vi "DisplayImage.vi"(0 "image color":T2, 1 "Image Pixel Data":u32[](array[numeric]), 3 "data type":T4(ring), 5 "Image grayscale":T2, 9 "width":u16, 11 "error in (no error)":errorcluster, 12 "height":u16, 13 "interpretation":T3(ring), 14 "bayer parameters":T1) -> (4 "display image":T2, 15 "error out":errorcluster)   [LabVIEW 2025, in "Automotive Vision UI.lvlib"]
doc: "Transform the received picture pixels to an actual image based on the image type."
uses:
  <vilib>/vision/Image Controls.llb/IMAQ Image.ctl
  Automotive Vision UI.lvlib
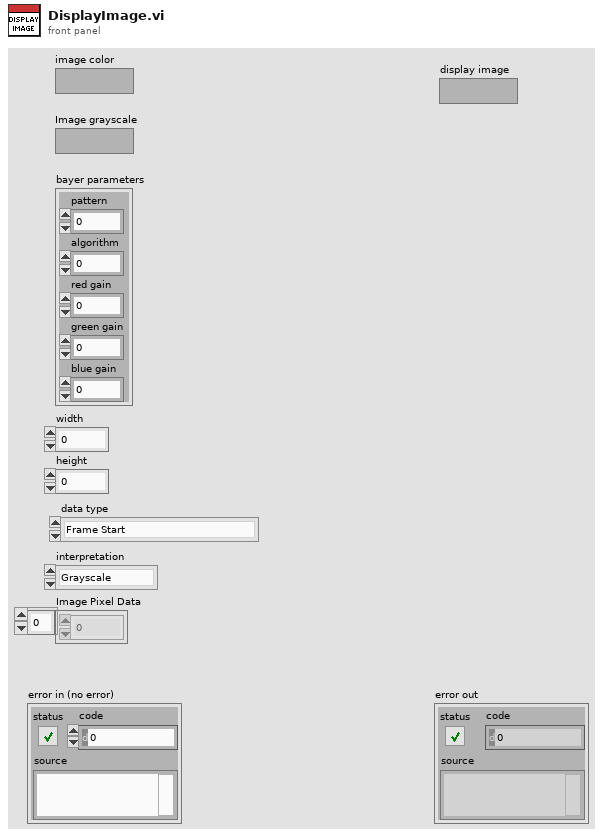
[diagram p1: front panel]
types:
  T1 = cluster{"pattern":i32, "algorithm":i32, "red gain":dbl, "green gain":dbl, "blue gain":dbl}
  T2 = typedef "IMAQ Image.ctl" = refnum<image>
  T3 = enum16{"Grayscale", "Bayer", "RGB", "YUV422", "YUV420", "Legacy YUV420"}
  T4 = enum8{"Frame Start", "Frame End", "Line Start", "Line End", "End of Transmission", "Reserved 0", "Reserved 1", "Reserved 2", "Generic Short Packet 1", "Generic Short Packet 2", "Generic Short Packet 3", "Generic Short Packet 4", "Generic Short Packet 5", "Generic Short Packet 6", "Generic Short Packet 7", "Generic Short Packet 8", "Null", "Blanking Data", "Embedded 8-bit non Image Data", "Generic Long Packet 1", "Generic Long Packet 2", "Generic Long Packet 3", "Generic Long Packet 4", "Reserved 3", "YUV420 8-bit", "YUV420 10-bit", "Legacy YUV420 8-bit", "Reserved 4", "YUV420 8-bit Chroma Shifted", "YUV420 10-bit Chroma Shifted", "YUV422 8-bit", "YUV422 10-bit", "RGB444", "RGB555", "RGB565", "RGB666", "RGB888", "Reserved 5", "Reserved 6", "RAW 24", "RAW 6", "RAW 7", "RAW 8", "RAW 10", "RAW 12", "RAW 14", "RAW 16", "RAW 20", "User Defined 8-bit Data 1", "User Defined 8-bit Data 2", "User Defined 8-bit Data 3", "User Defined 8-bit Data 4", "User Defined 8-bit Data 5", "User Defined 8-bit Data 6", "User Defined 8-bit Data 7", "User Defined 8-bit Data 8", "USL Command", "Reserved 7", "Reserved 8", "Reserved 9", "Reserved 10", "Reserved 11", "Reserved 12", "LRTE EPD Spacer"}
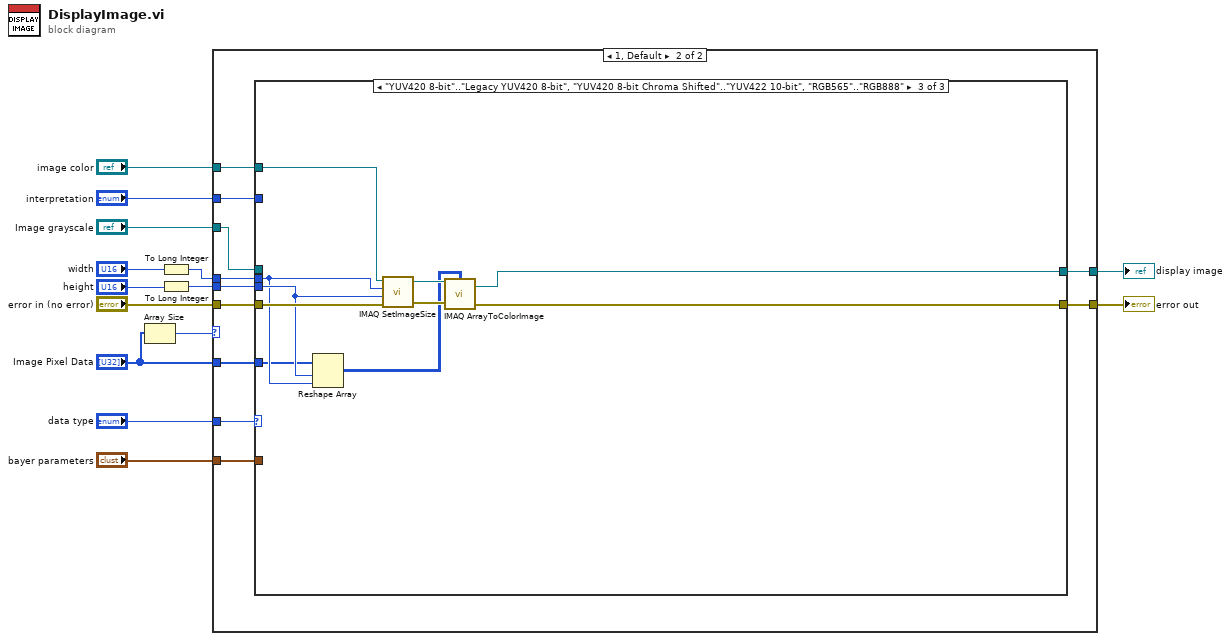
[diagram p0: block diagram]
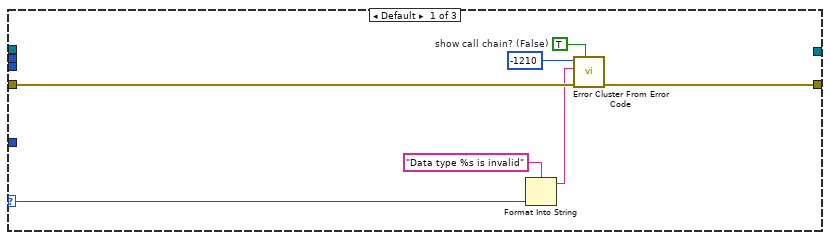
[diagram p3: hidden frame]
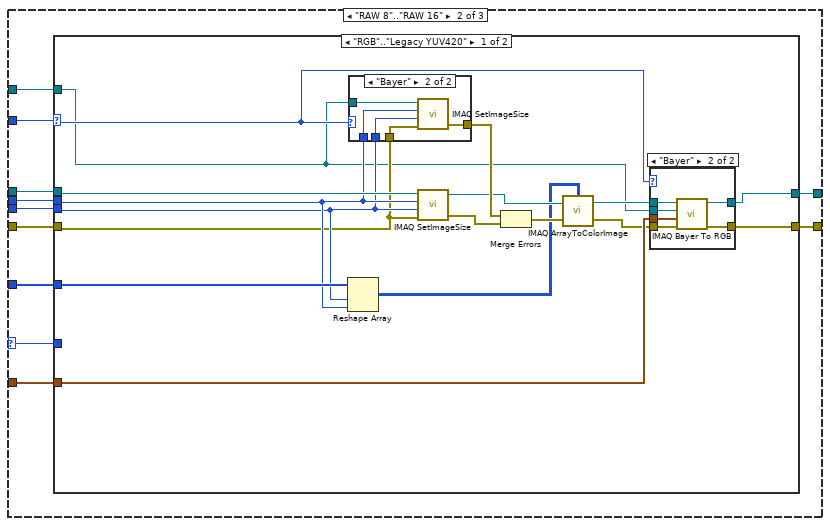
[diagram p4: hidden frame]
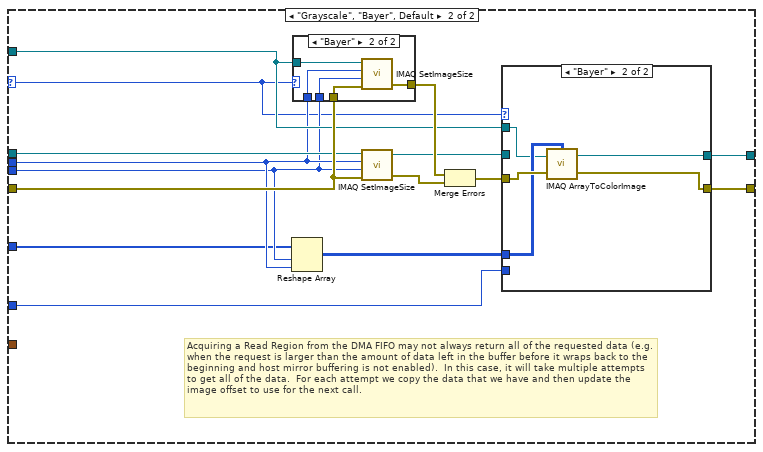
[diagram p7: hidden frame]
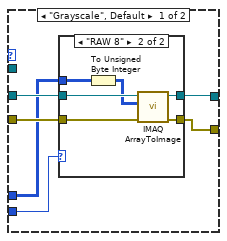
[diagram p8: hidden frame]
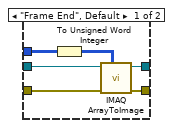
[diagram p9: hidden frame]
diagram:
  n1 = Array Size(array="Image Pixel Data") -> (size(s)=w1:i32)
  n2 = To Long Integer(number="width") -> (32bit integer=w12:i32)
  n3 = To Long Integer(number="height") -> (32bit integer=w13:i32)
  n4 = case shown="1, Default" w1 {
    tunnel: "error in (no error)" -> [w15 w27]
    tunnel: w13 -> [_ w26]
    tunnel: w12 -> [_ w25]
    tunnel: [w16 w24] -> w11
    tunnel: [w15 w23] -> w10
    tunnel: "data type" -> [_ w22]
    tunnel: "interpretation" -> [_ w21]
    tunnel: "image color" -> [_ w20]
    tunnel: "Image grayscale" -> [w16 w19]
    tunnel: "Image Pixel Data" -> [_ w18]
    tunnel: "bayer parameters" -> [_ w17]
    frame 0 {
    }
    frame 1, Default {
      n5 = case shown="\"YUV420 8-bit\"..\"Legacy YUV420 8-bit\", \"YUV420 8-bit Chroma Shifted\"..\"YUV422 10-bit\", \"RGB565\"..\"RGB888\"" w22 {
        selector: w22 -> [w28 w37 _]
        tunnel: w27 -> [w32 w45 w130]
        tunnel: w26 -> [_ w44 w129]
        tunnel: w25 -> [_ w43 w128]
        tunnel: [_ w42 w122] -> w24
        tunnel: [w31 w41 w121] -> w23
        tunnel: w21 -> [_ w40 _]
        tunnel: w20 -> [_ w39 w123]
        tunnel: w19 -> [_ w38 _]
        tunnel: w18 -> [_ w36 w127]
        tunnel: w17 -> [_ w35 _]
        frame Default {
          w33 = TRUE  # show call chain? (False)
          n6 = Format Into String(format string="Data type %s is invalid" ("error message (\"\")"), w28) -> (resulting string=w29:string)  [unwired: 2 in, 1 out]
          n7 = call <vilib>:"Error Cluster From Error Code.vi"("show call chain? (False)"=w33, "error in (no error)"=w32, "error message (\"\")"=w29, "error code (0)"=-1210) -> ("error out"=w31:errorcluster)  [unwired: 5 in]
        }
        frame "RAW 8".."RAW 16" {
          n8 = case shown="\"RGB\"..\"Legacy YUV420\"" w40 {
            selector: w40 -> [w55 w77]
            tunnel: w45 -> [w56 w90]
            tunnel: w44 -> [w57 w81]
            tunnel: w43 -> [w58 w82]
            tunnel: [w47 w88] -> w42
            tunnel: [w46 w87] -> w41
            tunnel: w39 -> [w48 w85]
            tunnel: w38 -> [w59 w86]
            tunnel: w37 -> [_ w79]
            tunnel: w36 -> [w60 w80]
            tunnel: w35 -> [w54 _]
            frame "RGB".."Legacy YUV420" {
              n9 = Reshape Array(w60, w57, w58) -> (w50:u32[][])
              n10 = case shown="\"Bayer\"" w55 {
                tunnel: w56 -> [w63 w68]
                tunnel: [w63 w67] -> w61
                tunnel: w48 -> [_ w66]
                tunnel: w57 -> [_ w65]
                tunnel: w58 -> [_ w64]
                frame "Grayscale", Default {
                }
                frame "Bayer" {
                  n11 = call "IMAQ SetImageSize"("error in (no error)"=w68, "Y Resolution"=w65, "X Resolution"=w64, "Image"=w66) -> ("error out"=w67:errorcluster)  [unwired: 1 in, 1 out]
                }
              }
              n12 = call "IMAQ SetImageSize"("error in (no error)"=w56, "Y Resolution"=w57, "X Resolution"=w58, "Image"=w59) -> ("error out"=w62:errorcluster, "Image Out"=w52:T2)  [unwired: 1 in]
              n13 = Merge Errors(w61, w62) -> (w51:errorcluster)
              n14 = call "IMAQ ArrayToColorImage"("Image Pixels (U32)"=w50, "Image"=w52, "error in (no error)"=w51) -> ("Image Out"=w53:T2, "error out"=w49:errorcluster)  [unwired: 2 in]
              n15 = case shown="\"Bayer\"" w55 {
                tunnel: w53 -> [w69 w76]
                tunnel: [w69 w75] -> w47
                tunnel: w49 -> [w70 w74]
                tunnel: [w70 w73] -> w46
                tunnel: w48 -> [_ w72]
                tunnel: w54 -> [_ w71]
                frame "Grayscale", Default {
                }
                frame "Bayer" {
                  n16 = call "IMAQ Bayer To RGB"("error in (no error)"=w74, "Bayer Parameters"=w71, "Image Dst"=w72, "Image Src"=w76) -> ("error out"=w73:errorcluster, "Image Dst Out"=w75:T2)  [unwired: 6 in]
                }
              }
            }
            frame "Grayscale", "Bayer", Default {
              # "Acquiring a Read Region from the DMA FIFO may not always return all of the requested data (e.g. when the request is larger than the amount of data left in the buffer before it wraps back to the beginning and host mirror buffering is not enabled).  In this case, it will take multiple attempts to get all of the data.  For each attempt we copy the data that we have and then update the image offset to use for the next call."
              n17 = Reshape Array(w80, w81, w82) -> (w78:u32[][])
              n18 = case shown="\"Bayer\"" w77 {
                tunnel: w90 -> [w115 w120]
                tunnel: [w115 w119] -> w89
                tunnel: w85 -> [_ w118]
                tunnel: w81 -> [_ w117]
                tunnel: w82 -> [_ w116]
                frame "Grayscale", Default {
                }
                frame "Bayer" {
                  n19 = call "IMAQ SetImageSize"("error in (no error)"=w120, "Y Resolution"=w117, "X Resolution"=w116, "Image"=w118) -> ("error out"=w119:errorcluster)  [unwired: 1 in, 1 out]
                }
              }
              n20 = call "IMAQ SetImageSize"("error in (no error)"=w90, "Y Resolution"=w81, "X Resolution"=w82, "Image"=w86) -> ("error out"=w91:errorcluster, "Image Out"=w84:T2)  [unwired: 1 in]
              n21 = Merge Errors(w89, w91) -> (w83:errorcluster)
              n22 = case shown="\"Bayer\"" w77 {
                tunnel: [w93 w112] -> w88
                tunnel: [w92 w111] -> w87
                tunnel: w85 -> [_ w110]
                tunnel: w84 -> [w97 _]
                tunnel: w83 -> [w96 w114]
                tunnel: w79 -> [w95 _]
                tunnel: w78 -> [w94 w113]
                frame "Grayscale", Default {
                  n23 = case shown="\"RAW 8\"" w95 {
                    tunnel: w97 -> [w103 w109]
                    tunnel: [w102 w108] -> w93
                    tunnel: w96 -> [w101 w107]
                    tunnel: [w100 w106] -> w92
                    tunnel: w94 -> [w99 w105]
                    frame "Frame End", Default {
                      n24 = To Unsigned Word Integer(number=w99) -> (unsigned 16bit integer=w98:u16[][])
                      n25 = call "IMAQ ArrayToImage"("Image Pixels (U16)"=w98, "error in (no error)"=w101, "Image"=w103) -> ("error out"=w100:errorcluster, "Image Out"=w102:T2)  [unwired: 7 in]
                    }
                    frame "RAW 8" {
                      n26 = To Unsigned Byte Integer(number=w105) -> (unsigned 8bit integer=w104:u8[][])
                      n27 = call "IMAQ ArrayToImage"("error in (no error)"=w107, "Image Pixels (U8)"=w104, "Image"=w109) -> ("error out"=w106:errorcluster, "Image Out"=w108:T2)  [unwired: 7 in]
                    }
                  }
                }
                frame "Bayer" {
                  n28 = call "IMAQ ArrayToColorImage"("Image Pixels (U32)"=w113, "Image"=w110, "error in (no error)"=w114) -> ("Image Out"=w112:T2, "error out"=w111:errorcluster)  [unwired: 2 in]
                }
              }
            }
          }
        }
        frame "YUV420 8-bit".."Legacy YUV420 8-bit", "YUV420 8-bit Chroma Shifted".."YUV422 10-bit", "RGB565".."RGB888" {
          n29 = Reshape Array(w127, w129, w128) -> (w124:u32[][])
          n30 = call "IMAQ SetImageSize"("error in (no error)"=w130, "Y Resolution"=w129, "X Resolution"=w128, "Image"=w123) -> ("error out"=w126:errorcluster, "Image Out"=w125:T2)  [unwired: 1 in]
          n31 = call "IMAQ ArrayToColorImage"("Image Pixels (U32)"=w124, "Image"=w125, "error in (no error)"=w126) -> ("Image Out"=w122:T2, "error out"=w121:errorcluster)  [unwired: 2 in]
        }
      }
    }
  }
  "display image" <- w11
  "error out" <- w10
